vi "Read protocols.vi"(8 "error in (no error)":errorcluster, 11 "ZM-CP-MX-multi_protocol in":refnum<class "ZM-CP-MX-multi_protocol.lvclass">) -> (0 "error out":errorcluster, 2 "ZM-CP-MX-PROTOCOLS":T1, 3 "ZM-CP-MX-multi_protocol out":refnum<class "ZM-CP-MX-multi_protocol.lvclass">)   [LabVIEW 2020, in "ZM-CP-MX-multi_protocol.lvlib" / "ZM-CP-MX-multi_protocol.lvclass"]
doc: "Reads one field of this class's private data. Generated by lvai_create_accessors from the class private data control."
uses:
  ZM-CP-MX-multi_protocol.lvclass
  ZM-CP-communication_protocol/ZM-CP-communication_protocol/ZM-CP-communication_protocol.lvclass
  ZM-CP-MX-multi_protocol.lvclass/ZM-CP-MX-multi_protocol.ctl
  ZM-CP-MX-PROTOCOLS.ctl
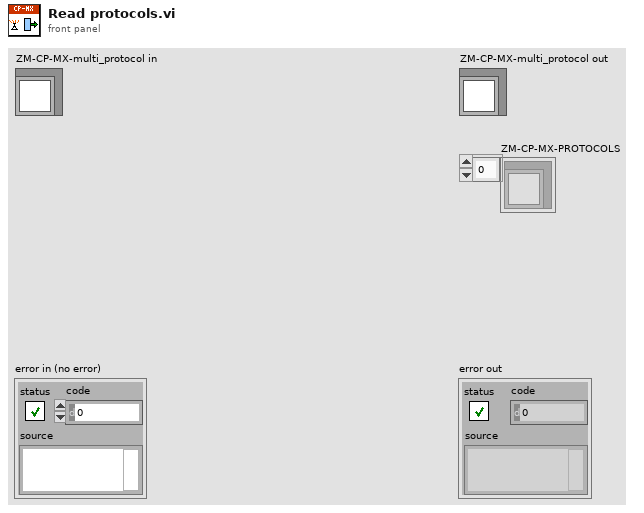
[diagram p1: front panel]
types:
  T1 = typedef "ZM-CP-MX-multi_protocol.lvlib/ZM-CP-MX-multi_protocol.lvclass/ZM-CP-MX-PROTOCOLS.ctl" = refnum<class "ZM-CP-communication_protocol.lvclass">[]
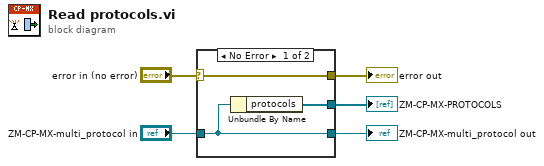
[diagram p0: block diagram]
diagram:
  n1 = case shown="No Error" "error in (no error)" {
    selector: "error in (no error)" -> [w8 w9]
    tunnel: [w8 w9] -> w4
    tunnel: [w7 w10] -> w2
    tunnel: "ZM-CP-MX-multi_protocol in" -> [w7 w10]
    tunnel: [w6 _] -> w1
    frame No Error {
      n2 = Unbundle By Name(w7) -> ("protocols"=w6:T1)
    }
    frame Error {
    }
  }
  "error out" <- w4
  "ZM-CP-MX-multi_protocol out" <- w2
  "ZM-CP-MX-PROTOCOLS" <- w1
